vi "Create OneOf Field Accessors.vi"(8 "error in (no error)":errorcluster, 10 "Message parameters":T1[](array[typedef]), 11 "Library in":refnum<vi>) -> (0 "error out":errorcluster, 3 "Library out":refnum<vi>)   [LabVIEW 2019, in "gRPC Template Creation Utility.lvlib"]
uses:
  gRPC Template Creation Utility.lvlib
  TypeDefs/Message Metadata (Scripting).ctl
  TypeDefs/Message Element Metadata (Scripting).ctl
  TypeDefs/Message Element Type.ctl
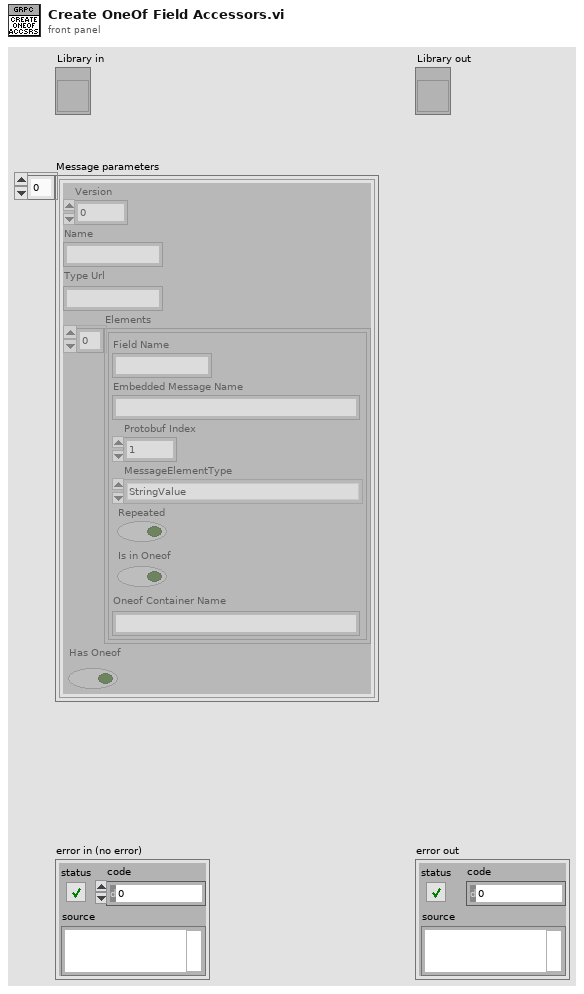
[diagram p1: front panel]
types:
  T1 = typedef "gRPC Template Creation Utility.lvlib/Message Metadata (Scripting).ctl" = cluster{"Version":i32, "Name":string, "Type Url":string, "Elements":T2[], "Has Oneof":bool}
  T2 = typedef "gRPC Template Creation Utility.lvlib/Message Element Metadata (Scripting).ctl" = cluster{"Field Name":string, "Embedded Message Name":string, "Protobuf Index":i32, "MessageElementType":T3, "Repeated":bool, "Is in Oneof":bool, "Oneof Container Name":string}
  T3 = typedef "gRPC Template Creation Utility.lvlib/Message Element Type.ctl" = enum32{"Int32Value", "FloatValue", "DoubleValue", "BoolValue", "StringValue", "MessageValue", "Int64Value", "UInt32Value", "UInt64Value", "EnumValue", "Bytes", "Fixed64", "Fixed32", "SFixed64", "SFixed32", "SInt64", "SInt32"}
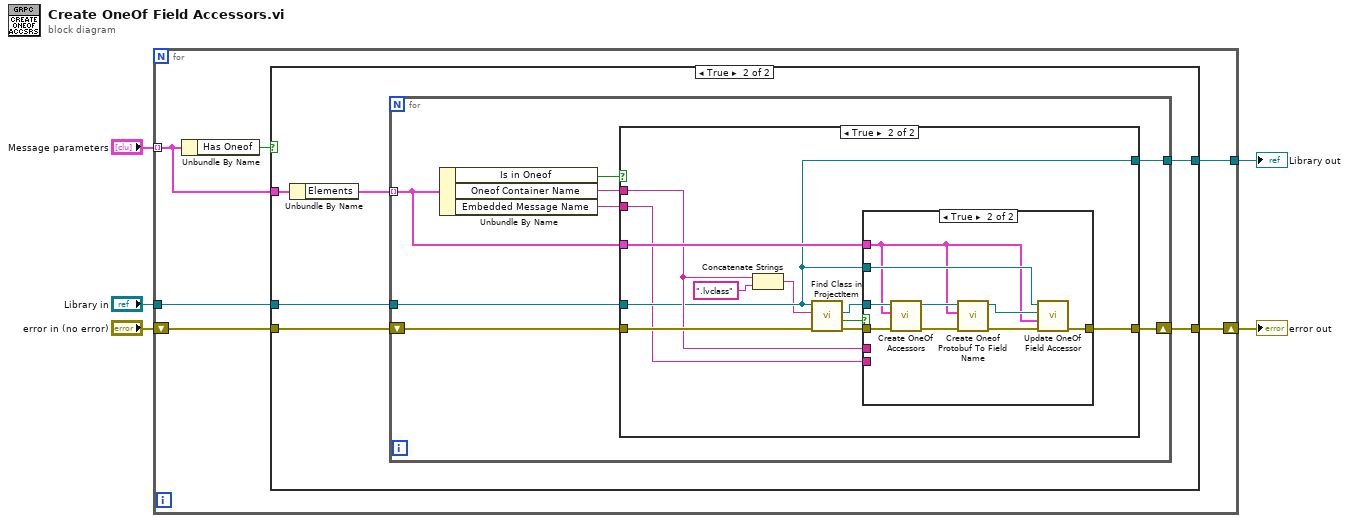
[diagram p0: block diagram]
diagram:
  n1 = for {
    tunnel: "Message parameters" -> [w10] mode=indexing
    tunnel: "Library in" -> [w8]
    shift-right: [w7] -> w2
    shift-left: "error in (no error)" -> [w9]
    tunnel: [w6] -> w1
    n2 = Unbundle By Name(w10) -> ("Has Oneof"=w11:bool)
    n3 = case shown="True" w11 {
      tunnel: w10 -> [_ w19]
      tunnel: w9 -> [w13 w17]
      tunnel: w8 -> [w12 w16]
      tunnel: [w13 w15] -> w7
      tunnel: [w12 w14] -> w6
      frame False {
      }
      frame True {
        n4 = Unbundle By Name(w19) -> ("Elements"=w18:T2[])
        n5 = for {
          tunnel: w18 -> [w27] mode=indexing
          tunnel: w16 -> [w25]
          shift-right: [w24] -> w15
          shift-left: w17 -> [w26]
          tunnel: [w23] -> w14
          n6 = Unbundle By Name(w27) -> ("Is in Oneof"=w22:bool, "Oneof Container Name"=w21:string, "Embedded Message Name"=w20:string)
          n7 = case shown="True" w22 {
            tunnel: w26 -> [w28 w38]
            tunnel: w27 -> [_ w40]
            tunnel: [w28 w39] -> w24
            tunnel: [w29 w33] -> w23
            tunnel: w21 -> [_ w36]
            tunnel: w25 -> [w29 w33]
            tunnel: w20 -> [_ w30]
            frame False {
            }
            frame True {
              n8 = Concatenate Strings(w36, ".lvclass" ("string")) -> (w32:string)
              n9 = call "Find Class in ProjectItem.vi"("error in (no error)"=w38, "Class Name"=w32, "ProjectItem in"=w33) -> ("error out"=w37:errorcluster, "Found?"=w35:bool, "LVClass out"=w34:refnum<vi>)  [unwired: 5 in, 1 out]
              n10 = case shown="True" w35 {
                tunnel: w40 -> [_ w42]
                tunnel: [w41 w43] -> w39
                tunnel: w37 -> [w41 w49]
                tunnel: w36 -> [_ _]
                tunnel: w34 -> [_ w48]
                tunnel: w33 -> [_ w45]
                tunnel: w30 -> [_ _]
                frame False {
                }
                frame True {
                  n11 = call "Create OneOf Accessors.vi"("error in (no error)"=w49, "MessageElementMetadata"=w42, "Oneof Class Ref In"=w48) -> ("error out"=w50:errorcluster, "Oneof Class Ref Out"=w44:refnum<vi>)  [unwired: 7 in]
                  n12 = call "Create Oneof Protobuf To Field Name.vi"("error in (no error)"=w50, "message element metadata"=w42, "class in"=w44) -> ("error out"=w47:errorcluster, "class out"=w46:refnum<vi>)  [unwired: 7 in]
                  n13 = call "Update OneOf Field Accessor.vi"("error in (no error)"=w47, "message element metadata"=w42, "class in"=w46, "library in"=w45) -> ("error out"=w43:errorcluster)  [unwired: 7 in]
                }
              }
            }
          }
        }
      }
    }
  }
  "error out" <- w2
  "Library out" <- w1
